vi "Add Cache Hints.vi"(8 "error in":errorcluster, 10 "method":string, 11 "response":string) -> (0 "error out":errorcluster, 3 "response out":string)   [LabVIEW 2020, in "MCP Server.lvlib"]
doc: "For the methods named in Cache Hints.vi, sets result.ttlMs and result.cacheScope of a JSON-RPC response (MCP 2026-07-28); for every other method response out is response unchanged. Used by Add Result Fields.vi.\n\nRuns regardless of error in, which is passed through unchanged; the JSONtext errors are not passed on."
uses:
  MCP Server.lvlib
  32540f87-00d8-434d-819b-fd8c8e3a5067.vi
  <vilib>/JDP Science/JSONtext/Variant to JSON Text.vi
  <vilib>/JDP Science/JSONtext/LVClass Serializer/JSONtext LVClass Serializer.lvclass
  <vilib>/JDP Science/JSONtext/JSONtext.lvlib
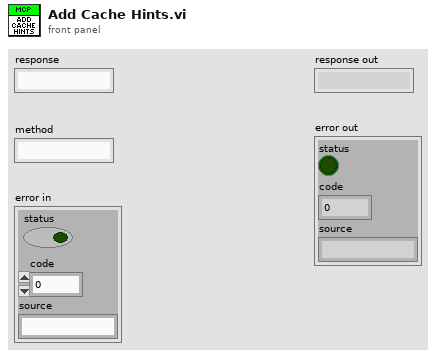
[diagram p1: front panel]
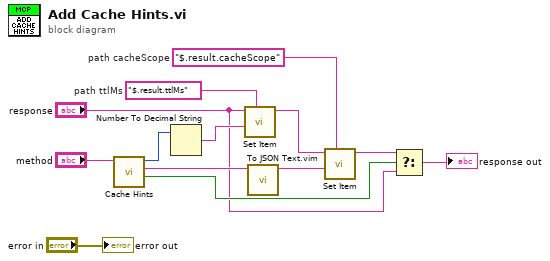
[diagram p0: block diagram]
diagram:
  w5 = "$.result.cacheScope"  # path cacheScope
  w4 = "$.result.ttlMs"  # path ttlMs
  n1 = call "Cache Hints.vi"("method"="method") -> ("cacheable?"=w6:bool, "cacheScope"=w7:string, "ttlMs"=w8:i32)  [unwired: 8 in]
  n2 = Number To Decimal String(number=w8) -> (decimal integer string=w9:string)  [unwired: 1 in]
  n3 = call <vilib>:"Set Item.vi"("$Path or Item Name"=w4, "JSON to Insert"=w9, "JSON"="response") -> ("<JSON>"=w11:string)  [unwired: 5 in, 2 out]
  n4 = call "To JSON Text.vim"("Anything"=w7) -> ("<JSON>"=w10:string)  [unwired: 9 in, 1 out]
  n5 = call <vilib>:"Set Item.vi"("$Path or Item Name"=w5, "JSON to Insert"=w10, "JSON"=w11) -> ("<JSON>"=w12:string)  [unwired: 5 in, 2 out]
  n6 = Select(t=w12, s=w6, f="response") -> (s? t:f=→"response out":string)
  "error out" <- "error in"
